vi "CSE ISP - config file.vi"(6 "cmd":enum16{"load", "save"}(ring), 7 "Ctrl refnums":refnum<vi>[](array[refnum]), 8 "error in":errorcluster, 10 "forced saving":bool, 11 "ISP menu":refnum<k9>) -> (0 "error out":errorcluster, 3 "dup ISP menu":refnum<k9>)   [LabVIEW 2021]
doc: "::: CalcExpress Toolkit :::\nCopyright (c) 2000-2026 Konstantin Shifershteyn. All rights reserved."
uses:
  <vilib>/Utility/sysdir.llb/System Directory Type.ctl
  <vilib>/Utility/config.llb/NI_LVConfig.lvlib
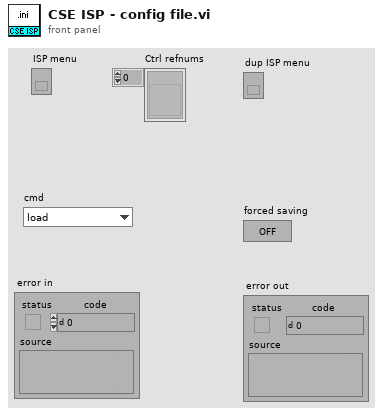
[diagram p1: front panel]
types:
  T1 = typedef "System Directory Type.ctl" = i32
  T2 = enum32{"invalid OS target", "Mac OS", "Windows 3.1", "Windows 95/NT", "Solaris 1", "Solaris 2", "HP-UX", "PowerMAX", "Linux", "Irix", "Rhapsody", "BeOS", "AIX", "OSF1", "VxWorks", "PharLap", "Carbon", "RTX", "Windows x64", "Linux x64", "Mac OS X x64"}
  T3 = typedef "NI_LVConfig.lvlib/Config Data RefNum.ctl" = refnum<k1>
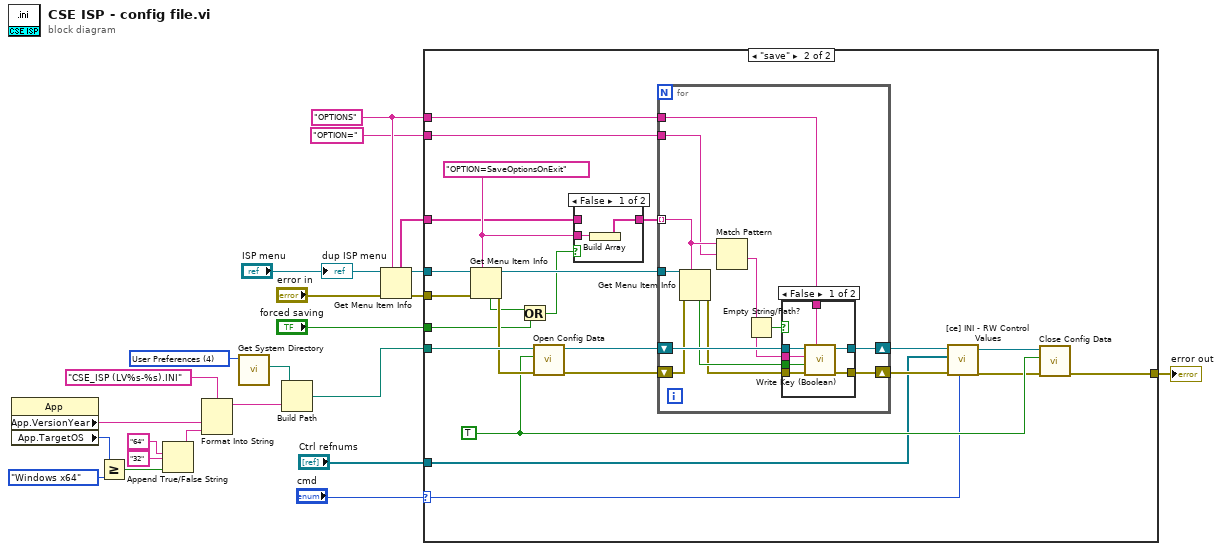
[diagram p0: block diagram]
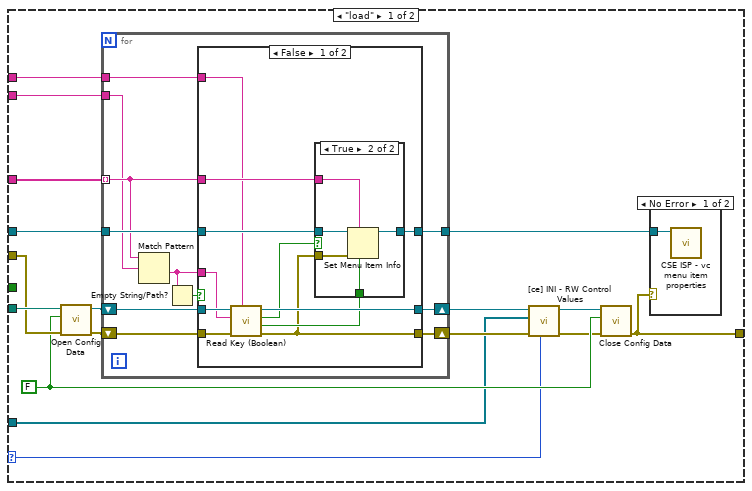
[diagram p2: hidden frame]
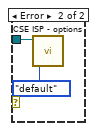
[diagram p3: hidden frame]
diagram:
  w5 = T1 4 items=["User Home"=0, "User Desktop"=1, "User Documents"=2, "User Application Data"=3, "User Preferences"=4, "User Temporary"=5, "Public Documents"=6, "Public Application Data"=7, "Public Preferences"=8, "Public Cache"=13, "System Core Libraries"=9, "System Installed Libraries"=10, "Application Files"=11, "Boot Volume Root"=12] ("system directory type")
  w20 = "OPTIONS" ("item tag")
  n1 = property class="App"() -> ("App.VersionYear"=w11:string, "App.TargetOS"=w9:T2)  [unwired: 2 in, 2 out]
  n2 = Greater Or Equal?(x=w9, y=T2."Windows x64" ("Application:Target:Operating System")) -> (x >= y?=w10:bool)
  n3 = Append True/False String(1:w10, 2:"32", 3:"64") -> (0:w8:string)  [unwired: 1 in]
  n4 = Format Into String(format string="CSE_ISP (LV%s-%s).INI", w11, w8) -> (resulting string=w6:string)  [unwired: 2 in, 1 out]
  n5 = call <vilib>:"Get System Directory.vi"("system directory type"=w5) -> ("system directory"=w7:path)  [unwired: 10 in]
  n6 = Build Path(base path=w7, name or relative path=w6) -> (appended path=w14:path)
  n7 = Get Menu Item Info(7:w20, 8:"error in", 11:"ISP menu") -> (0:w18:errorcluster, 3:w22:refnum<k9>, 5:w23:string[])  [unwired: 4 out]
  n8 = case shown="\"save\"" "cmd" {
    selector: "cmd" -> [w24 w75]
    tunnel: w23 -> [w40 w94]
    tunnel: w22 -> [w39 w97]
    tunnel: w14 -> [w36 w96]
    tunnel: w20 -> [w35 w86]
    tunnel: w18 -> [w34 w89]
    tunnel: [w31 w87] -> w17
    tunnel: "OPTION=" ("item tag") -> [w33 w85]
    tunnel: "forced saving" -> [_ w84]
    tunnel: "Ctrl refnums" -> [w25 w76]
    frame "load" {
      w30 = FALSE ("create file if necessary? (T)")
      n9 = call <vilib>:"Open Config Data.vi"("error in (no error)"=w34, "create file if necessary (T)"=w30, "configuration file path"=w36) -> ("error out"=w37:errorcluster, "refnum"=w38:T3)  [unwired: 6 in, 1 out]
      n10 = for {
        shift-right: [w53] -> w29
        shift-left: w38 -> [w54]
        shift-right: [w50] -> w27
        shift-left: w37 -> [w52]
        tunnel: w40 -> [w49] mode=indexing
        tunnel: w39 -> [w51]
        tunnel: w35 -> [w44]
        tunnel: w33 -> [w46]
        tunnel: [w45] -> w32
        n11 = Match Pattern(string=w49, regular expression=w46) -> (after substring=w47:string)  [unwired: 1 in, 3 out]
        n12 = Empty String/Path?(string/path=w47) -> (empty?=w48:bool)
        n13 = case shown="False" w48 {
          tunnel: w54 -> [w65 w74]
          tunnel: [w64 w74] -> w53
          tunnel: w52 -> [w63 w73]
          tunnel: w51 -> [w61 w72]
          tunnel: [w60 w73] -> w50
          tunnel: w47 -> [w59 _]
          tunnel: w49 -> [w58 _]
          tunnel: [w57 w72] -> w45
          tunnel: w44 -> [w56 _]
          frame False {
            n14 = call <vilib>:"Read Key (Boolean).vi"("section"=w56, "error in (no error)"=w63, "key"=w59, "refnum"=w65) -> ("error out"=w60:errorcluster, "value"=w62:bool, "found?"=w55:bool, "refnum out"=w64:T3)  [unwired: 4 in]
            n15 = case shown="True" w55 {
              tunnel: w62 -> [_ w71]
              tunnel: w61 -> [w66 w70]
              tunnel: w60 -> [_ w69]
              tunnel: w58 -> [_ w68]
              tunnel: [w66 w67] -> w57
              frame False {
              }
              frame True {
                n16 = Set Menu Item Info(6:w71, 7:w68, 8:w69, 11:w70) -> (3:w67:refnum<k9>)  [unwired: 3 in, 1 out]
              }
            }
          }
          frame True {
          }
        }
      }
      n17 = call "[ce] INI - RW Control Values.vi"("cmd (load)"=w24, "error in"=w27, "Ctrl refnums"=w25, "INI refnum"=w29) -> ("error out"=w26:errorcluster, "dup INI refnum"=w28:T3)  [unwired: 6 in]
      n18 = call <vilib>:"Close Config Data.vi"("error in (no error)"=w26, "write file if changed (T)"=w30, "refnum"=w28) -> ("error out"=w31:errorcluster)  [unwired: 7 in, 1 out]
      n19 = case shown="No Error" w31 {
        tunnel: w32 -> [w41 w43]
        frame No Error {
          n20 = call "CSE ISP - vc menu item properties.vi"("ISP menu"=w41) -> ()  [unwired: 7 in, 2 out]
        }
        frame Error {
          n21 = call "CSE ISP - options.vi"("cmd"=enum16{"get", "default"}."default", "ISP menu"=w43) -> ()  [unwired: 2 in, 8 out]
        }
      }
    }
    frame "save" {
      w81 = TRUE
      w95 = "OPTION=SaveOptionsOnExit" ("item tag")
      n22 = Get Menu Item Info(7:w95, 8:w89, 11:w97) -> (0:w88:errorcluster, 3:w90:refnum<k9>, 4:w83:bool)  [unwired: 4 out]
      n23 = Or(x=w83, y=w84) -> (x .or. y?=w82:bool)
      n24 = call <vilib>:"Open Config Data.vi"("error in (no error)"=w88, "create file if necessary (T)"=w81, "configuration file path"=w96) -> ("error out"=w92:errorcluster, "refnum"=w93:T3)  [unwired: 6 in, 1 out]
      n25 = case shown="False" w82 {
        tunnel: w95 -> [w120 _]
        tunnel: [w119 w121] -> w91
        tunnel: w94 -> [_ w121]
        frame False {
          n26 = Build Array(w120) -> (w119:string[])
        }
        frame True {
        }
      }
      n27 = for {
        shift-right: [w103] -> w80
        shift-left: w93 -> [w107]
        shift-right: [w102] -> w78
        shift-left: w92 -> [w105]
        tunnel: w91 -> [w108] mode=indexing
        tunnel: w90 -> [w109]
        tunnel: w86 -> [w101]
        tunnel: w85 -> [w98]
        n28 = Get Menu Item Info(7:w108, 8:w105, 11:w109) -> (0:w104:errorcluster, 4:w106:bool)  [unwired: 5 out]
        n29 = Match Pattern(string=w108, regular expression=w98) -> (after substring=w100:string)  [unwired: 1 in, 3 out]
        n30 = Empty String/Path?(string/path=w100) -> (empty?=w99:bool)
        n31 = case shown="False" w99 {
          tunnel: w107 -> [w116 w118]
          tunnel: w106 -> [w115 _]
          tunnel: w100 -> [w114 _]
          tunnel: w104 -> [w113 w117]
          tunnel: [w112 w118] -> w103
          tunnel: [w111 w117] -> w102
          tunnel: w101 -> [w110 _]
          frame False {
            n32 = call <vilib>:"Write Key (Boolean).vi"("section"=w110, "error in (no error)"=w113, "value"=w115, "key"=w114, "refnum"=w116) -> ("error out"=w111:errorcluster, "refnum out"=w112:T3)  [unwired: 4 in, 1 out]
          }
          frame True {
          }
        }
      }
      n33 = call "[ce] INI - RW Control Values.vi"("cmd (load)"=w75, "error in"=w78, "Ctrl refnums"=w76, "INI refnum"=w80) -> ("error out"=w77:errorcluster, "dup INI refnum"=w79:T3)  [unwired: 6 in]
      n34 = call <vilib>:"Close Config Data.vi"("error in (no error)"=w77, "write file if changed (T)"=w81, "refnum"=w79) -> ("error out"=w87:errorcluster)  [unwired: 7 in, 1 out]
    }
  }
  "error out" <- w17
  "dup ISP menu" <- "ISP menu"
